vi "Make Output Schema.vi"(8 "error in":errorcluster, 10 "terminals":T1(array[cluster]), 11 "outputs":T2(array[cluster])) -> (0 "error out":errorcluster, 3 "output schema":string)   [LabVIEW 2020, in "MCP Server.lvlib"]
doc: "Makes the outputSchema of a tool, for Complete Tool Entry.vi: an object schema with one property per output that is not a picture, named like the outputs in structuredContent and in the text of tools/call, and all of them in required. Each property comes from Make Output Property Schema.vi. A tool without such outputs gets an empty output schema."
uses:
  MCP Server.lvlib
  d0ba5213-9537-43b8-81e0-165763c4dde1.vi
  <vilib>/JDP Science/JSONtext/Variant to JSON Text.vi
  <vilib>/JDP Science/JSONtext/support/Format JSON Object.vi
  <vilib>/JDP Science/JSONtext/LVClass Serializer/JSONtext LVClass Serializer.lvclass
  <vilib>/JDP Science/JSONtext/JSONtext.lvlib
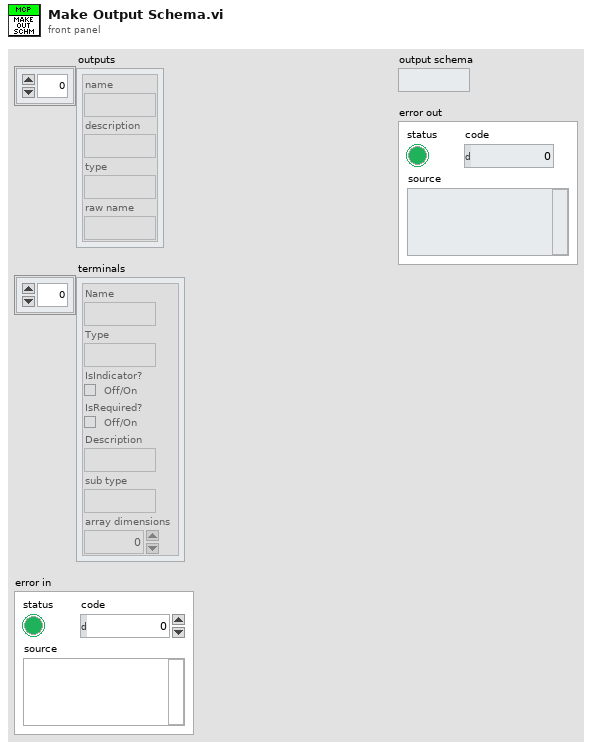
[diagram p1: front panel]
types:
  T1 = cluster{"Name":string, "Type":string, "IsIndicator?":bool, "IsRequired?":bool, "Description":string, "sub type":string, "array dimensions":i32}[]
  T2 = cluster{"name":string, "description":string, "type":string, "raw name":string}[]
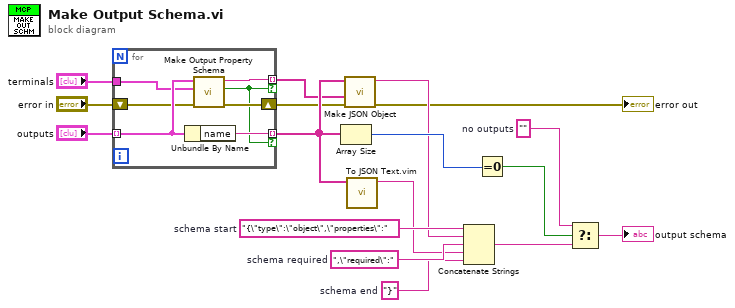
[diagram p0: block diagram]
diagram:
  w5 = ""  # no outputs
  w6 = "}"  # schema end
  w8 = ",\"required\":"  # schema required
  w10 = "{\"type\":\"object\",\"properties\":"  # schema start
  n1 = for {
    tunnel: "outputs" -> [w24] mode=indexing
    tunnel: "terminals" -> [w23]
    shift-right: [w22] -> w12
    shift-left: "error in" -> [w21]
    tunnel: [w20] -> w14 mode=indexing if=w19
    tunnel: [w18] -> w13 mode=indexing if=w19
    n2 = Unbundle By Name(w24) -> ("name"=w20:string)
    n3 = call "Make Output Property Schema.vi"("error in"=w21, "terminals"=w23, "output"=w24) -> ("error out"=w22:errorcluster, "listed?"=w19:bool, "property schema"=w18:string)  [unwired: 6 in]
  }
  n4 = Array Size(array=w14) -> (size(s)=w11:i32)
  n5 = call <vilib>:"Make JSON Object.vi"("error in (no error)"=w12, "JSON Items"=w13, "Item Names"=w14) -> ("error out"=→"error out":errorcluster, "<JSON>"=w9:string)  [unwired: 7 in]
  n6 = call "To JSON Text.vim"("Anything"=w14) -> ("<JSON>"=w7:string)  [unwired: 9 in, 1 out]
  n7 = Concatenate Strings(w10, w9, w8, w7, w6) -> (w3:string)
  n8 = Equal To 0?(x=w11) -> (x = 0?=w4:bool)
  n9 = Select(t=w5, s=w4, f=w3) -> (s? t:f=→"output schema":string)
